vi "SQL_Example_1.vi"() -> ()   [LabVIEW 2024]
uses:
  DB-Tool.lvlib
panel:
  out "No User Right":bool
  out "Server Connection OK":bool
  out "Fehler Connection":errorcluster
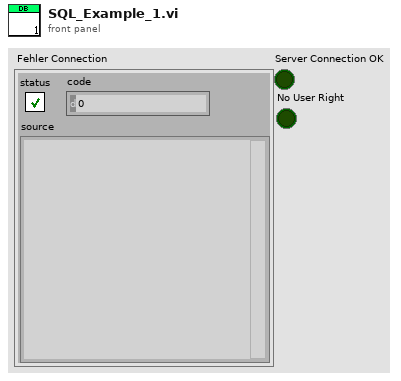
[diagram p1: front panel]
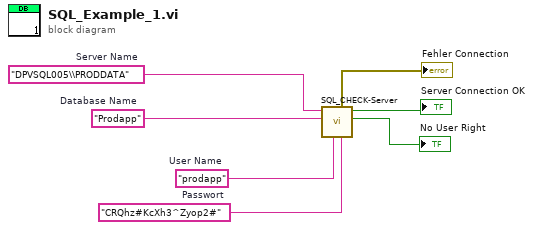
[diagram p0: block diagram]
diagram:
  w1 = "CRQhz#KcXh3^Zyop2#"  # Passwort
  w2 = "prodapp"  # User Name
  w7 = "Prodapp"  # Database Name
  w3 = "DPVSQL005\\PRODDATA"  # Server Name
  n1 = call "SQL_CHECK-Server.vi"("Passwort"=w1, "User Name"=w2, "Database Name"=w7, "Server Name"=w3) -> ("No User Right"=→"No User Right":bool, "Server Connection OK"=→"Server Connection OK":bool, "Fehler Connection"=→"Fehler Connection":errorcluster)  [unwired: 3 in, 2 out]
